vi "Exit.vi"(8 "error in (no error)":errorcluster, 11 "Ready in":refnum<class "Ready.lvclass">) -> (0 "error out":errorcluster, 3 "Ready out":refnum<class "Ready.lvclass">)   [LabVIEW 2014, in "States.lvlib" / "Ready.lvclass"]
doc: "This override sends a Log Event message to the UI, with the string \"Exiting Idle State\" as its payload."
uses:
  Ready.lvclass
  Process State/CoordinatorState.lvclass
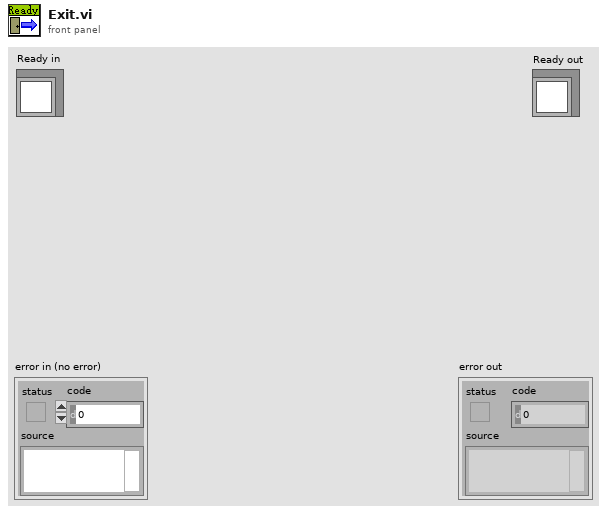
[diagram p1: front panel]
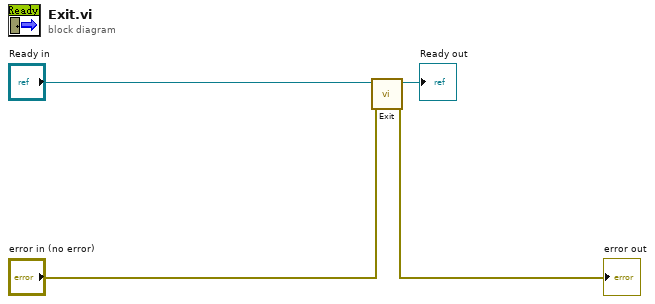
[diagram p0: block diagram]
diagram:
  n1 = call-parent "Exit.vi"("error in (no error)"="error in (no error)", "Old State"="Ready in") -> ("error out"=→"error out":errorcluster, "New State"=→"Ready out":refnum<class "Ready.lvclass">)  [unwired: 8 in]
